vi "Upload TDMS Metadata.vi"(8 "error in (no error)":errorcluster, 9 "Run ID":string, 10 "TDMS File":path, 11 "Sift TDMS Uploader in":refnum<class "Sift TDMS Uploader.lvclass">) -> (0 "error out":errorcluster, 3 "Sift TDMS Uploader out":refnum<class "Sift TDMS Uploader.lvclass">)   [LabVIEW 2024, in "Sift TDMS Uploader.lvlib" / "Sift TDMS Uploader.lvclass"]
uses:
  Sift TDMS Uploader.lvclass
  <vilib>/addons/_JKI.lib/REST Client/classes/REST Client/HTTP Header.ctl
  <vilib>/NI/Advanced HTTP Client/Header--Combo Box.ctl
  Types/Metadata Number.ctl
  Types/Metadata Key.ctl
  Types/Metadata Boolean.ctl
  Types/Metadata String.ctl
  Sift TDMS Uploader.lvclass/Sift TDMS Uploader.ctl
  <vilib>/Utility/error.llb/Error Cluster From Error Code.vi
  <vilib>/ErrorRing/Error Ring.xnode
  <vilib>/addons/_JKI.lib/REST Client/classes/REST Client/REST Client.lvclass
  <vilib>/addons/_JKI.lib/Serialization/JSON/JKI JSON Serialization.lvlib
  <vilib>/Utility/Data Type/NI_Data Type.lvlib
  <userlib>/_OpenG.lib/error/error.llb/openg_error.lvlib
  <vilib>/NI/Advanced HTTP Client/Session.lvclass
  Sift TDMS Uploader.lvlib
panel:
  in  "Metadata String":T1={"key"={"name"="", "type"=enum."METADATA_KEY_TYPE_STRING"}, "stringValue"=""}
  in  "Metadata Boolean":T3={"key"={"name"="", "type"=enum."METADATA_KEY_TYPE_BOOLEAN"}, "booleanValue"=FALSE}
  in  "Metadata Number":T4={"key"={"name"="", "type"=enum."METADATA_KEY_TYPE_NUMBER"}, "numberValue"=0.0}
  out "Response body":string
  in  "User-Agent Header":T5={"header"="User-Agent", "value"="labview"}
  in  "Authorization Header":T5={"header"="Authorization", "value"=""}
  out "Request JSON":string
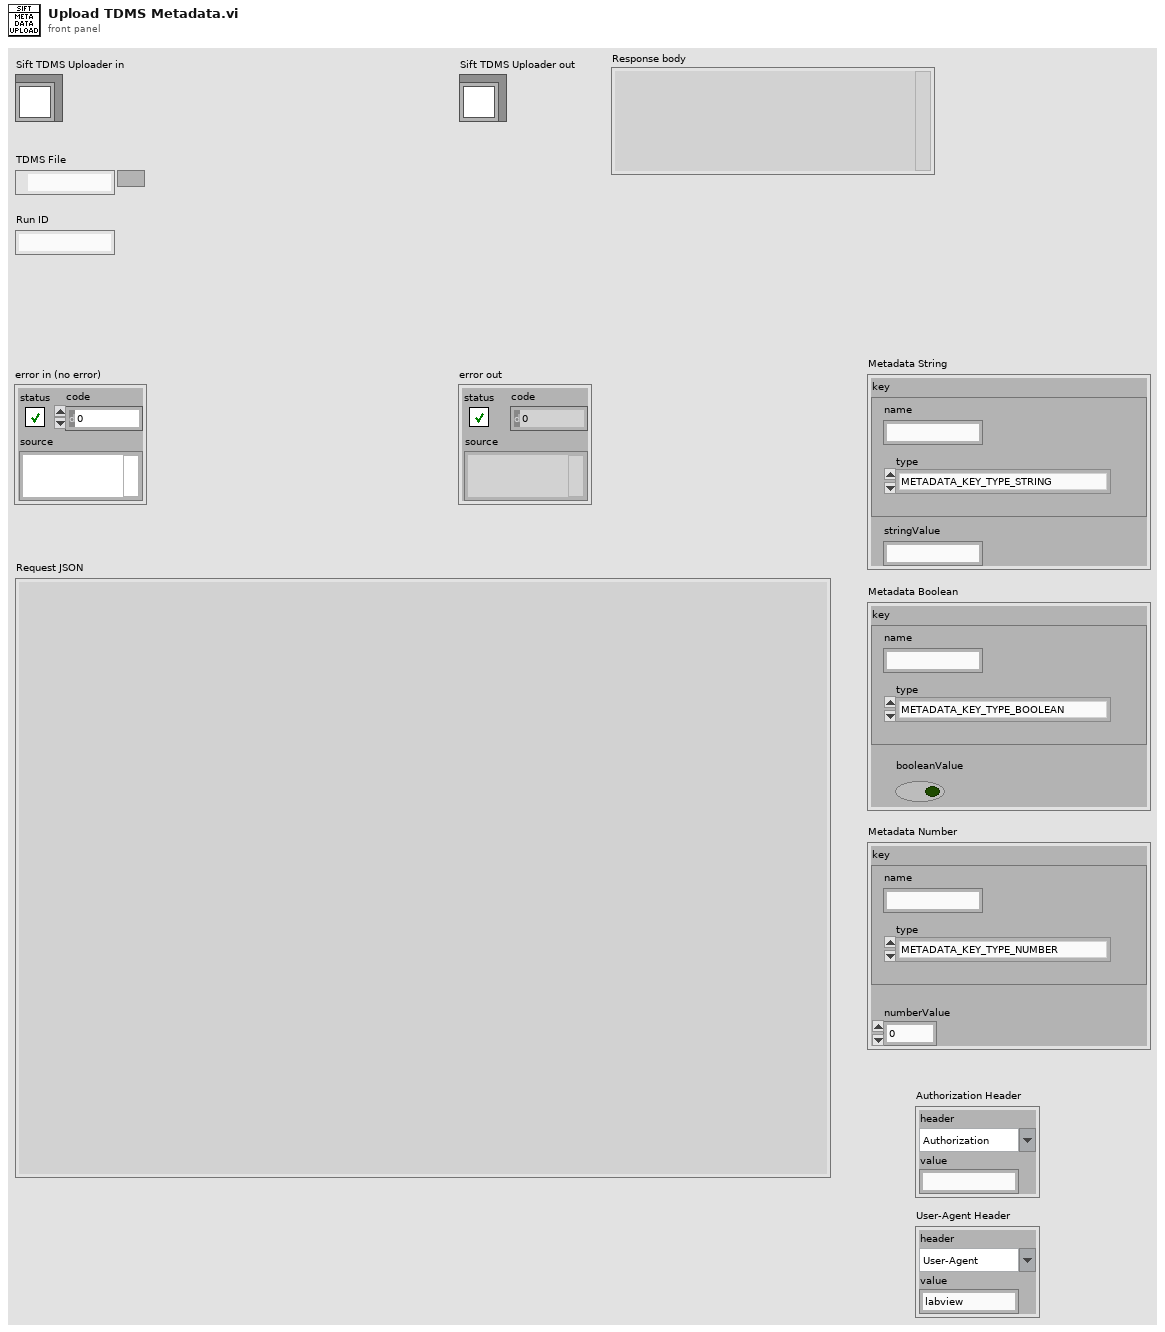
[diagram p1: front panel]
types:
  T1 = typedef "Sift TDMS Uploader.lvlib/Metadata String.ctl" = cluster{"key":T2, "stringValue":string}
  T2 = typedef "Sift TDMS Uploader.lvlib/Metadata Key.ctl" = cluster{"name":string, "type":enum16{"METADATA_KEY_TYPE_UNSPECIFIED", "METADATA_KEY_TYPE_BOOLEAN", "METADATA_KEY_TYPE_NUMBER", "METADATA_KEY_TYPE_STRING"}}
  T3 = typedef "Sift TDMS Uploader.lvlib/Metadata Boolean.ctl" = cluster{"key":T2, "booleanValue":bool}
  T4 = typedef "Sift TDMS Uploader.lvlib/Metadata Number.ctl" = cluster{"key":T2, "numberValue":dbl}
  T5 = typedef "REST Client.lvlib/REST Client.lvclass/HTTP Header.ctl" = cluster{"header":T6, "value":string}
  T6 = typedef "lib_NI_Advanced HTTP Client.lvlib/Session.lvclass/Header--Combo Box.ctl" = string
  T7 = cluster{"run":cluster{"runId":string, "metadata":variant[]}, "updateMask":string}
  T8 = typedef "NI_Data Type.lvlib/Data Type.ctl" = enum8{"Invalid Type", "Void", "I8", "I16", "I32", "I64", "U8", "U16", "U32", "U64", "Single Float", "Double Float", "Extended Float", "Single Complex", "Double Complex", "Extended Complex", "Enum U8", "Enum U16", "Enum U32", "Enum U64", "Single Float With Unit", "Double Float With Unit", "Extended Float With Unit", "Single Complex with Unit", "Double Complex with Unit", "Extended Complex with Unit", "Boolean", "String", "Path", "Picture", "Tag", "Array", "Cluster", "Variant", "LV Variant", "Waveform", "Timestamp", "Digital Waveform", "Digital Data", "ExpressData", "Refnum", "External Data", "VI", "Poly VI", "LabVIEW Class Instance", "Fixed Point", "Set Collection", "Map Collection"}
  T9 = typedef "LVNumericRepresentation.ctl" = enum32{"Extended Precision", "Double Precision", "Single Precision", "Long", "Word", "Byte", "Unsigned Long", "Unsigned Word", "Unsigned Byte", "Complex Extended", "Complex Double", "Complex Single", "Quad", "Unsigned Quad", "Fixed-Point"}
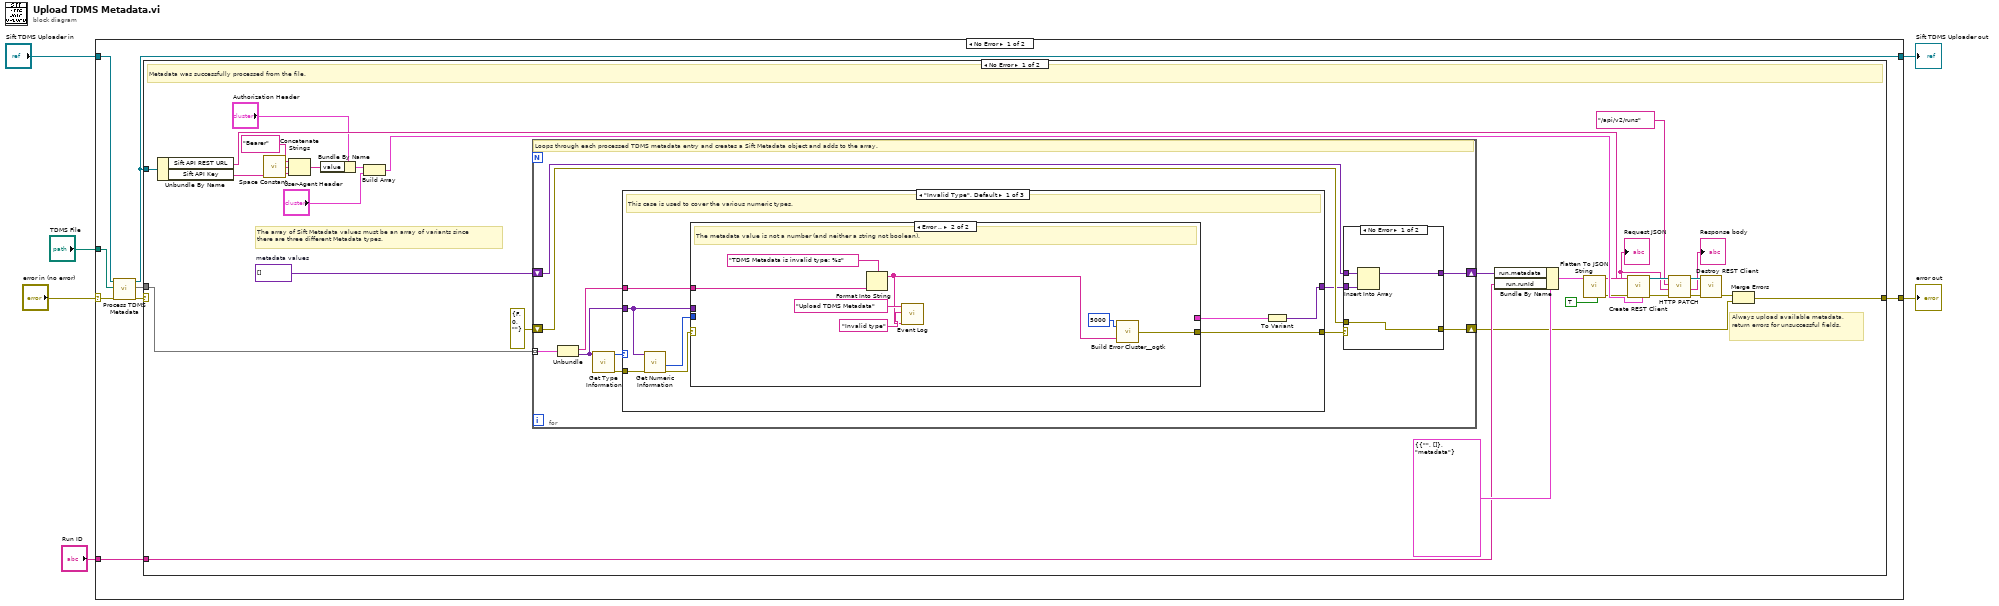
[diagram p0: block diagram]
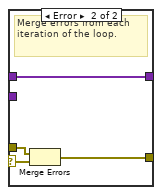
[diagram p2: hidden frame]
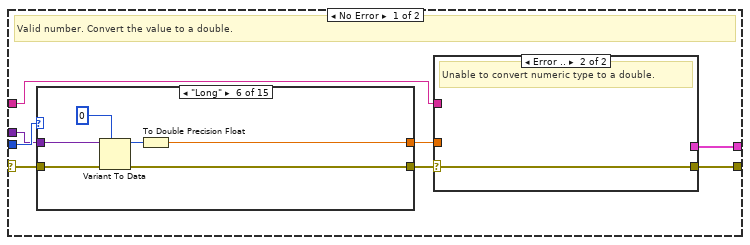
[diagram p3: hidden frame]
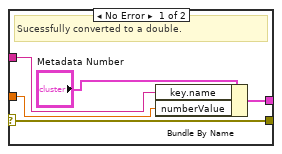
[diagram p4: hidden frame]
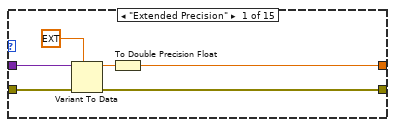
[diagram p5: hidden frame]
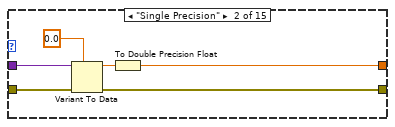
[diagram p6: hidden frame]
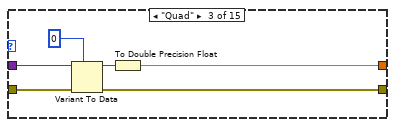
[diagram p7: hidden frame]
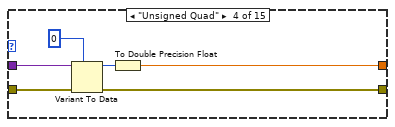
[diagram p8: hidden frame]
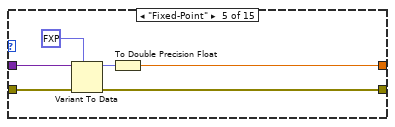
[diagram p9: hidden frame]
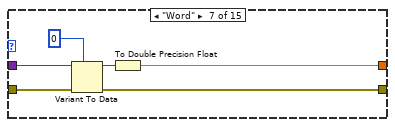
[diagram p10: hidden frame]
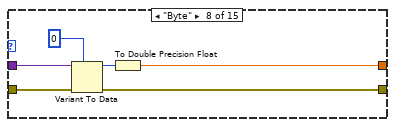
[diagram p11: hidden frame]
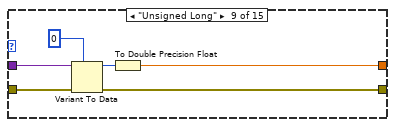
[diagram p12: hidden frame]
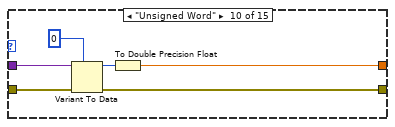
[diagram p13: hidden frame]
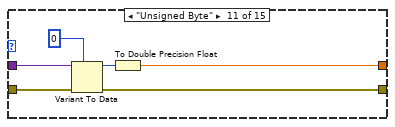
[diagram p14: hidden frame]
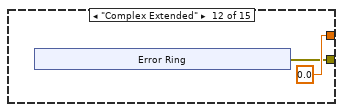
[diagram p15: hidden frame]
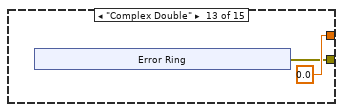
[diagram p16: hidden frame]
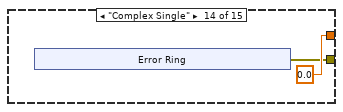
[diagram p17: hidden frame]
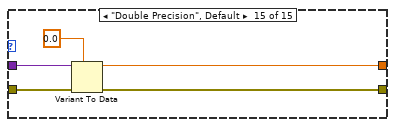
[diagram p18: hidden frame]
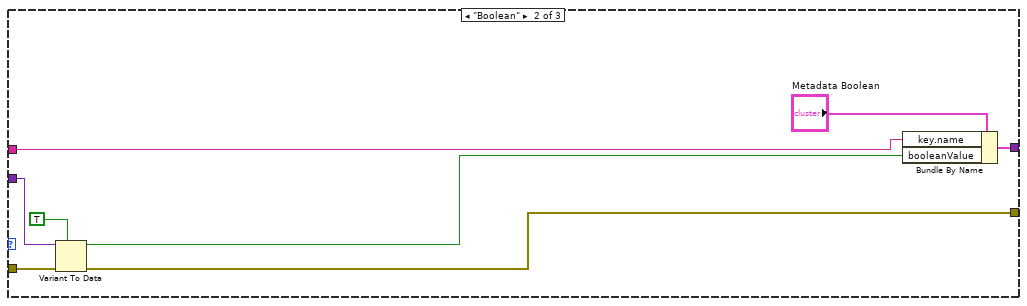
[diagram p19: hidden frame]
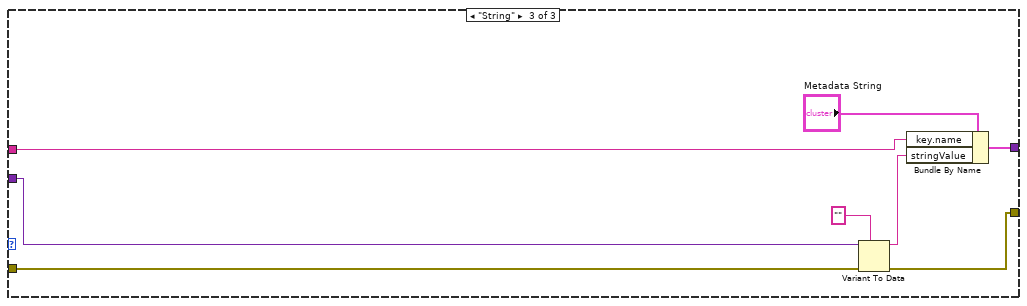
[diagram p20: hidden frame]
diagram:
  n1 = case shown="No Error" "error in (no error)" {
    selector: "error in (no error)" -> [w12 w202]
    tunnel: [w8 w202] -> w5
    tunnel: [w11 w201] -> w3
    tunnel: "Sift TDMS Uploader in" -> [w14 w201]
    tunnel: "TDMS File" -> [w13 _]
    tunnel: "Run ID" -> [w9 _]
    frame No Error {
      n2 = call-dynamic "Process TDMS Metadata.vi"("Sift TDMS Uploader in"=w14, "TDMS File"=w13, "error in (no error)"=w12) -> ("Sift TDMS Uploader out"=w11:refnum<class "Sift TDMS Uploader.lvclass">, "Metadata"=w10:map{string, variant}, "error out"=w7:errorcluster)  [unwired: 5 in]
      n3 = case shown="No Error" w7 {
        selector: w7 -> [_ w200]
        tunnel: w11 -> [w42 _]
        tunnel: w10 -> [w29 _]
        tunnel: w9 -> [w26 _]
        tunnel: [w15 w200] -> w8
        frame No Error {
          w28 = variant[] []  # metadata values
          # "Always upload available metadata, \nreturn errors for unsuccessful fields."
          # "The array of Sift Metadata values must be an array of variants since\nthere are three different Metadata types."
          # "Metadata was successfully processed from the file."
          n4 = Unbundle By Name(w42) -> ("Sift API REST URL"=w39:string, "Sift API Key"=w32:string)
          n5 = call <vilib>:"Space Constant.vi"() -> ("String"=w31:string)
          n6 = Concatenate Strings("Bearer", w31, w32) -> (w35:string)
          n7 = Bundle By Name(cluster="Authorization Header", "value"=w35) -> (w34:T5)
          n8 = Build Array(w34, "User-Agent Header") -> (w33:T5[])
          n9 = for {
            tunnel: w29 -> [w54] mode=indexing
            shift-right: [w44] -> w27
            shift-left: w28 -> [w46]
            shift-right: [w47] -> w17
            shift-left: errorcluster {"status"=FALSE, "code"=0, "source"=""} ("error in (no error)") -> [w48]
            # "Loops through each processed TDMS metadata entry and creates a Sift Metadata object and adds to the array."
            n10 = Unbundle(w54) -> (w52:string, w51:variant)
            n11 = call <vilib>:"Get Type Information.vi"("variant"=w51) -> ("error out"=w50:errorcluster, "type"=w53:T8)  [unwired: 6 in, 3 out]
            n12 = case shown="\"Invalid Type\", Default" w53 {
              tunnel: w52 -> [w65 w184 w192]
              tunnel: w51 -> [w66 w189 w199]
              tunnel: w50 -> [w70 w188 w195]
              tunnel: [w68 w187 w196] -> w49
              tunnel: [w63 w186 w194] -> w45
              frame "Invalid Type", Default {
                # "This case is used to cover the various numeric types."
                n13 = call <vilib>:"Get Numeric Information.vi"("error in (no error)"=w70, "variant"=w66) -> ("error out"=w69:errorcluster, "representation"=w67:T9)  [unwired: 6 in, 2 out]
                n14 = case shown="Error .." w69 {
                  selector: w69 -> [w76 _]
                  tunnel: [w74 w177] -> w68
                  tunnel: w67 -> [w78 _]
                  tunnel: w66 -> [w77 _]
                  tunnel: w65 -> [w72 w181]
                  tunnel: [w71 _] -> w64
                  frame No Error {
                    # "Valid number. Convert the value to a double."
                    n15 = case shown="\"Long\"" w78 {
                      tunnel: w77 -> [w89 w95 w101 w107 w113 w119 w125 w131 w137 w143 w149 _ _ _ w175]
                      tunnel: w76 -> [w88 w94 w100 w106 w112 w118 w124 w130 w136 w142 w148 _ _ _ w174]
                      tunnel: [w87 w93 w99 w105 w111 w117 w123 w129 w135 w141 w147 w151 w158 w165 w173] -> w75
                      tunnel: [w85 w91 w97 w103 w109 w115 w121 w127 w133 w139 w145 0.0 0.0 0.0 w172] -> w73
                      frame "Extended Precision" {
                        n16 = Variant To Data(error in=w88, type=ext 0.0, Variant=w89) -> (data=w86:ext, error out=w87:errorcluster)
                        n17 = To Double Precision Float(number=w86) -> (double precision float=w85:dbl)
                      }
                      frame "Single Precision" {
                        n18 = Variant To Data(error in=w94, type=sgl 0.0, Variant=w95) -> (data=w92:sgl, error out=w93:errorcluster)
                        n19 = To Double Precision Float(number=w92) -> (double precision float=w91:dbl)
                      }
                      frame "Quad" {
                        n20 = Variant To Data(error in=w100, type=i64 0, Variant=w101) -> (data=w98:i64, error out=w99:errorcluster)
                        n21 = To Double Precision Float(number=w98) -> (double precision float=w97:dbl)
                      }
                      frame "Unsigned Quad" {
                        n22 = Variant To Data(error in=w106, type=u64 0, Variant=w107) -> (data=w104:u64, error out=w105:errorcluster)
                        n23 = To Double Precision Float(number=w104) -> (double precision float=w103:dbl)
                      }
                      frame "Fixed-Point" {
                        n24 = Variant To Data(error in=w112, type=fxp<+,1,1> 0.0, Variant=w113) -> (data=w110:fxp<+,1,1>, error out=w111:errorcluster)
                        n25 = To Double Precision Float(number=w110) -> (double precision float=w109:dbl)
                      }
                      frame "Long" {
                        n26 = Variant To Data(error in=w118, type=0, Variant=w119) -> (data=w116:i32, error out=w117:errorcluster)
                        n27 = To Double Precision Float(number=w116) -> (double precision float=w115:dbl)
                      }
                      frame "Word" {
                        n28 = Variant To Data(error in=w124, type=i16 0, Variant=w125) -> (data=w122:i16, error out=w123:errorcluster)
                        n29 = To Double Precision Float(number=w122) -> (double precision float=w121:dbl)
                      }
                      frame "Byte" {
                        n30 = Variant To Data(error in=w130, type=i8 0, Variant=w131) -> (data=w128:i8, error out=w129:errorcluster)
                        n31 = To Double Precision Float(number=w128) -> (double precision float=w127:dbl)
                      }
                      frame "Unsigned Long" {
                        n32 = Variant To Data(error in=w136, type=u32 0, Variant=w137) -> (data=w134:u32, error out=w135:errorcluster)
                        n33 = To Double Precision Float(number=w134) -> (double precision float=w133:dbl)
                      }
                      frame "Unsigned Word" {
                        n34 = Variant To Data(error in=w142, type=u16 0, Variant=w143) -> (data=w140:u16, error out=w141:errorcluster)
                        n35 = To Double Precision Float(number=w140) -> (double precision float=w139:dbl)
                      }
                      frame "Unsigned Byte" {
                        n36 = Variant To Data(error in=w148, type=u8 0, Variant=w149) -> (data=w146:u8, error out=w147:errorcluster)
                        n37 = To Double Precision Float(number=w146) -> (double precision float=w145:dbl)
                      }
                      frame "Complex Extended" {
                        n38 = xnode "Error Ring"() -> ("error out"=w151:errorcluster)
                      }
                      frame "Complex Double" {
                        n39 = xnode "Error Ring"() -> ("error out"=w158:errorcluster)
                      }
                      frame "Complex Single" {
                        n40 = xnode "Error Ring"() -> ("error out"=w165:errorcluster)
                      }
                      frame "Double Precision", Default {
                        n41 = Variant To Data(error in=w174, type=0.0, Variant=w175) -> (data=w172:dbl, error out=w173:errorcluster)
                      }
                    }
                    n42 = case shown="Error .." w75 {
                      selector: w75 -> [w83 w84]
                      tunnel: [w83 w84] -> w74
                      tunnel: w73 -> [w82 _]
                      tunnel: w72 -> [w79 _]
                      tunnel: [w81 _] -> w71
                      frame No Error {
                        # "Sucessfully converted to a double."
                        n43 = Bundle By Name(cluster="Metadata Number", "key.name"=w79, "numberValue"=w82) -> (w81:T4)
                      }
                      frame Error {
                        # "Unable to convert numeric type to a double."
                      }
                    }
                  }
                  frame Error {
                    # "The metadata value is not a number (and neither a string not boolean)."
                    n44 = Format Into String(format string="TDMS Metadata is invalid type: %s" ("initial string"), w181) -> (resulting string=w178:string)  [unwired: 2 in, 1 out]
                    n45 = call "Event Log.vi"("Message"=w178, "Event Type"="Invalid type", "Location"="Upload TDMS Metadata") -> ()  [unwired: 9 in]
                    n46 = call <userlib>:"Build Error Cluster__ogtk.vi"("String to Prepend to source (\"\")"=w178, "code"=5000) -> ("error out"=w177:errorcluster)
                  }
                }
                n47 = To Variant(anything=w64) -> (Variant=w63:variant)
              }
              frame "Boolean" {
                n48 = Variant To Data(error in=w188, type=TRUE, Variant=w189) -> (data=w190:bool, error out=w187:errorcluster)
                n49 = Bundle By Name(cluster="Metadata Boolean", "key.name"=w184, "booleanValue"=w190) -> (w186:T3)
              }
              frame "String" {
                n50 = Variant To Data(error in=w195, type="", Variant=w199) -> (data=w197:string, error out=w196:errorcluster)
                n51 = Bundle By Name(cluster="Metadata String", "key.name"=w192, "stringValue"=w197) -> (w194:T1)
              }
            }
            n52 = case shown="No Error" w49 {
              selector: w49 -> [_ w62]
              tunnel: w48 -> [w58 w61]
              tunnel: [w58 w60] -> w47
              tunnel: w46 -> [w57 w59]
              tunnel: w45 -> [w56 _]
              tunnel: [w55 w59] -> w44
              frame No Error {
                n53 = Insert Into Array(array=w57, new element=w56) -> (w55:variant[])  [unwired: 1 in]
              }
              frame Error {
                # "Merge errors from each iteration of the loop."
                n54 = Merge Errors(w61, w62) -> (w60:errorcluster)
              }
            }
          }
          n55 = Bundle By Name(cluster=T7 {"run"={"runId"="", "metadata"=[]}, "updateMask"="metadata"}, "run.metadata"=w27, "run.runId"=w26) -> (w25:T7)
          n56 = call <vilib>:"Flatten To JSON String.vi"("Enums As String (F)"=TRUE, "Variant"=w25) -> ("error out"=w24:errorcluster, "JSON String"=w22:string)  [unwired: 8 in]
          "Request JSON" <- w22
          n57 = call <vilib>:"Create REST Client.vi"("Default Headers ([JSON])"=w33, "error in (no error)"=w24, "Base URL"=w39) -> ("error out"=w41:errorcluster, "REST Client out"=w38:refnum<class "REST Client.lvclass">)  [unwired: 7 in]
          n58 = call-dynamic "HTTP PATCH.vi"("error in (no error)"=w41, "Request body"=w22, "Path"="/api/v2/runs", "REST Client in"=w38) -> ("error out"=w40:errorcluster, "Response body"=→"Response body":string, "REST Client out"=w37:refnum<class "REST Client.lvclass">)  [unwired: 2 in, 3 out]
          n59 = call-dynamic "Destroy REST Client.vi"("error in (no error)"=w40, "REST Client in"=w37) -> ("error out"=w16:errorcluster)  [unwired: 9 in]
          n60 = Merge Errors(w16, w17) -> (w15:errorcluster)
        }
        frame Error {
          # "Metadata was not sucessfully processed from the file."
        }
      }
    }
    frame Error {
    }
  }
  "error out" <- w5
  "Sift TDMS Uploader out" <- w3
